vi "Test Measurement Iterations.vi"() -> (0 "error out":errorcluster)   [LabVIEW 2026, in "Measurement Test Harness.lvclass"]
doc: "ITER-001/002/003: increment and completion boundary; reset preserves requested count and identity."
uses:
  fixtures/Measurement Test Harness/Measurement Test Harness.lvclass
  fixtures/Measurement Test Harness/Measurement Test Harness.lvclass/Measurement Test Harness.ctl
  <vilib>/addons/_JKI Toolkits/Caraya/classes/Test/Test.lvclass
  source/framework/Measurement Actor/Measurement.lvclass
  <vilib>/addons/_JKI Toolkits/Caraya/classes/Assert/Assert.lvclass
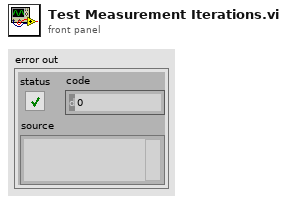
[diagram p1: front panel]
types:
  T1 = typedef "Measurement Actor.lvlib/Measurement.lvclass/Iteration count.ctl" = cluster{"Desired Iterations":i32, "Current":i32}
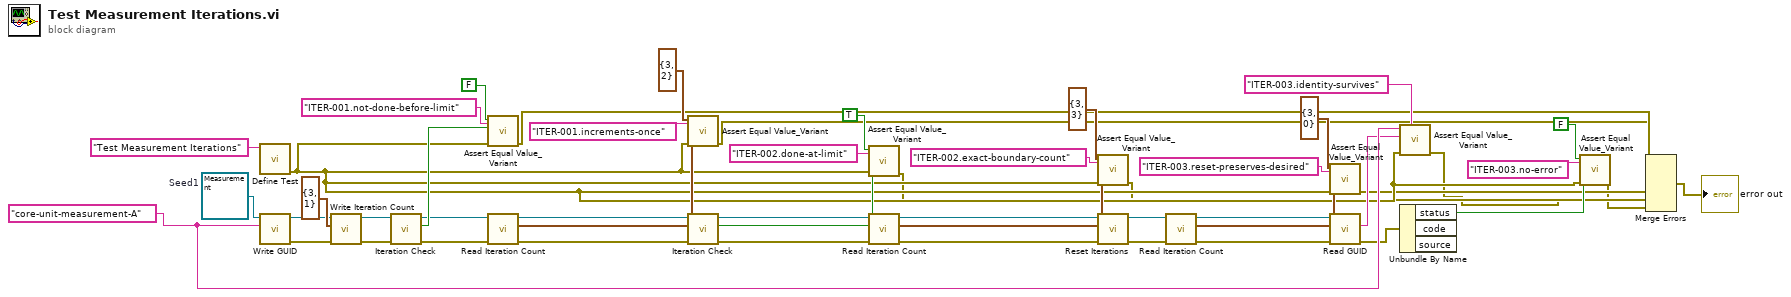
[diagram p0: block diagram]
diagram:
  w16 = "core-unit-measurement-A"
  w49 = refnum<class "Measurement.lvclass"> refnum  # Seed1
  n1 = call <vilib>:"Define Test.vi"("Label (VI Title)"="Test Measurement Iterations") -> ("error out"=w12:errorcluster)  [unwired: 9 in, 1 out]
  n2 = call "Write GUID.vi"("GUID"=w16, "Measurement in"=w49) -> ("error out"=w48:errorcluster, "Measurement out"=w46:refnum<class "Measurement.lvclass">)  [unwired: 8 in]
  n3 = call "Write Iteration Count.vi"("error in (no error)"=w48, "Iteration Count"=cluster{"Desired Iterations":i32, "Current":i32} {"Desired Iterations"=3, "Current"=1}, "Measurement in"=w46) -> ("error out"=w44:errorcluster, "Measurement out"=w45:refnum<class "Measurement.lvclass">)  [unwired: 7 in]
  n4 = call "Iteration Check.vi"("error in (no error)"=w44, "Measurement in"=w45) -> ("error out"=w39:errorcluster, "Done?"=w42:bool, "Measurement out"=w40:refnum<class "Measurement.lvclass">)  [unwired: 7 in]
  n5 = call <vilib>:"Assert Equal Value_Variant.vi"("Label"="ITER-001.not-done-before-limit", "error in (no error)"=w12, "Actual"=w42, "Expected"=FALSE) -> ("error out"=w8:errorcluster)  [unwired: 6 in, 1 out]
  n6 = call "Read Iteration Count.vi"("error in (no error)"=w39, "Measurement in"=w40) -> ("error out"=w34:errorcluster, "Iteration Count"=w37:T1, "Measurement out"=w35:refnum<class "Measurement.lvclass">)  [unwired: 7 in]
  n7 = call <vilib>:"Assert Equal Value_Variant.vi"("Label"="ITER-001.increments-once", "error in (no error)"=w12, "Actual"=w37, "Expected"=cluster{"Desired Iterations":i32, "Current":i32} {"Desired Iterations"=3, "Current"=2}) -> ("error out"=w7:errorcluster)  [unwired: 6 in, 1 out]
  n8 = call "Iteration Check.vi"("error in (no error)"=w34, "Measurement in"=w35) -> ("error out"=w29:errorcluster, "Done?"=w32:bool, "Measurement out"=w30:refnum<class "Measurement.lvclass">)  [unwired: 7 in]
  n9 = call <vilib>:"Assert Equal Value_Variant.vi"("Label"="ITER-002.done-at-limit", "error in (no error)"=w12, "Actual"=w32, "Expected"=TRUE) -> ("error out"=w6:errorcluster)  [unwired: 6 in, 1 out]
  n10 = call "Read Iteration Count.vi"("error in (no error)"=w29, "Measurement in"=w30) -> ("error out"=w24:errorcluster, "Iteration Count"=w27:T1, "Measurement out"=w25:refnum<class "Measurement.lvclass">)  [unwired: 7 in]
  n11 = call <vilib>:"Assert Equal Value_Variant.vi"("Label"="ITER-002.exact-boundary-count", "error in (no error)"=w12, "Actual"=w27, "Expected"=cluster{"Desired Iterations":i32, "Current":i32} {"Desired Iterations"=3, "Current"=3}) -> ("error out"=w5:errorcluster)  [unwired: 6 in, 1 out]
  n12 = call "Reset Iterations.vi"("error in (no error)"=w24, "Measurement in"=w25) -> ("error out"=w22:errorcluster, "Measurement out"=w23:refnum<class "Measurement.lvclass">)  [unwired: 8 in]
  n13 = call "Read Iteration Count.vi"("error in (no error)"=w22, "Measurement in"=w23) -> ("error out"=w17:errorcluster, "Iteration Count"=w20:T1, "Measurement out"=w18:refnum<class "Measurement.lvclass">)  [unwired: 7 in]
  n14 = call <vilib>:"Assert Equal Value_Variant.vi"("Label"="ITER-003.reset-preserves-desired", "error in (no error)"=w12, "Actual"=w20, "Expected"=cluster{"Desired Iterations":i32, "Current":i32} {"Desired Iterations"=3, "Current"=0}) -> ("error out"=w4:errorcluster)  [unwired: 6 in, 1 out]
  n15 = call "Read GUID.vi"("error in (no error)"=w17, "Measurement in"=w18) -> ("error out"=w13:errorcluster, "GUID"=w15:string)  [unwired: 7 in, 1 out]
  n16 = call <vilib>:"Assert Equal Value_Variant.vi"("Label"="ITER-003.identity-survives", "error in (no error)"=w12, "Actual"=w15, "Expected"=w16) -> ("error out"=w3:errorcluster)  [unwired: 6 in, 1 out]
  n17 = Unbundle By Name(w13) -> ("status"=w10:bool)  [unwired: 2 out]
  n18 = call <vilib>:"Assert Equal Value_Variant.vi"("Label"="ITER-003.no-error", "error in (no error)"=w12, "Actual"=w10, "Expected"=FALSE) -> ("error out"=w2:errorcluster)  [unwired: 6 in, 1 out]
  n19 = Merge Errors(w8, w7, w6, w5, w4, w3, w2) -> (→"error out":errorcluster)
